vi "Remove Buffer.vi"(8 "error in":errorcluster, 9 "Name":string, 11 "BufferMap in":refnum<data-value>) -> (0 "error out":errorcluster, 2 "Buffer":refnum<data-value>, 3 "BufferMap":refnum<data-value>)   [LabVIEW 2013, in "CircularBuffer.lvlib" / "VariantBufferMap.lvclass"]
doc: "This VI writes one data element into the current location in the buffer. The location in the buffer is updated automatically."
uses:
  VariantBufferMap.lvclass
  VariantBuffer/VariantBuffer.lvclass
  VariantBufferMap.lvclass/VariantBufferMap.ctl
  VariantBuffer/WriteBufferError.vi
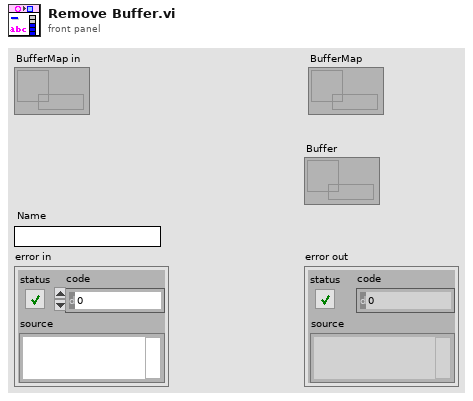
[diagram p1: front panel]
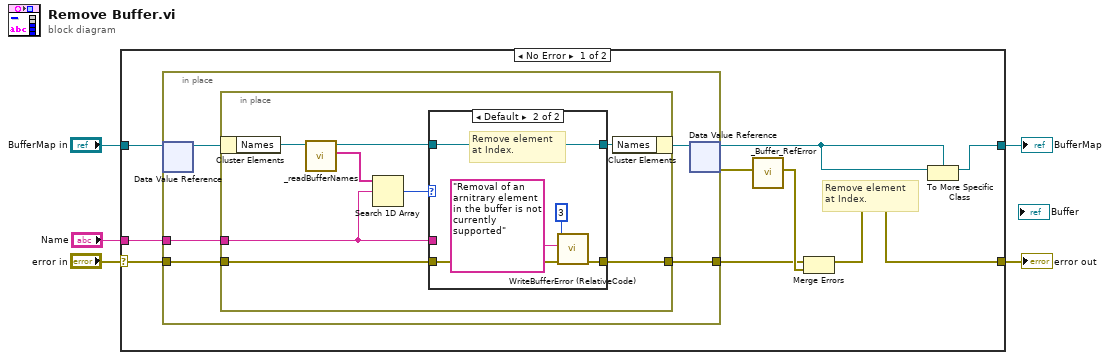
[diagram p0: block diagram]
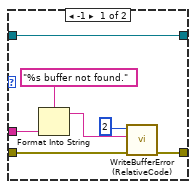
[diagram p2: hidden frame]
diagram:
  n1 = case shown="No Error" "error in" {
    selector: "error in" -> [w9 w41]
    tunnel: "BufferMap in" -> [w12 w40]
    tunnel: [w13 w40] -> w4
    tunnel: [w6 w41] -> w3
    tunnel: "Name" -> [w14 _]
    frame No Error {
      # "Remove element \nat Index."
      n2 = in-place {
        in-place-border: w14 -> [w17]
        in-place-border: [w16] -> w8
        in-place-border: w9 -> [w15]
        n3 = in-place-dvr #1(w12) -> (w19:refnum<class "VariantBufferMap.lvclass">)  [unwired: 1 out]
        n4 = in-place {
          in-place-border: w17 -> [w25]
          in-place-border: [w24] -> w16
          in-place-border: w15 -> [w20]
          n5 = in-place-cluster #2(w19) -> ("Names"=w27:refnum<data-value>)
          n6 = call "_readBufferNames.vi"("Data Value Reference in"=w27) -> ("Names"=w23:string[], "Data Value Reference out"=w21:refnum<data-value>)  [unwired: 9 in]
          n7 = Search 1D Array(1D array=w23, element=w25) -> (index of element=w22:i32)  [unwired: 1 in]
          n8 = case shown="Default" w22 {
            tunnel: w21 -> [w34 w39]
            tunnel: [w34 w39] -> w26
            tunnel: w25 -> [w30 _]
            tunnel: [w33 w37] -> w24
            tunnel: w20 -> [w31 w38]
            frame -1 {
              n9 = Format Into String(format string="%s buffer not found." ("error message (\"\")"), w30) -> (resulting string=w29:string)  [unwired: 2 in, 1 out]
              n10 = call "WriteBufferError (RelativeCode).vi"("error in (no error)"=w31, "Error message"=w29, "Relative error code (548600 + input)"=2 ("error code (0)")) -> ("error out"=w33:errorcluster)  [unwired: 8 in]
            }
            frame Default {
              # "Remove element \nat Index."
              n11 = call "WriteBufferError (RelativeCode).vi"("error in (no error)"=w38, "Error message"="Removal of an arnitrary element in the buffer is not currently supported" ("error message (\"\")"), "Relative error code (548600 + input)"=3) -> ("error out"=w37:errorcluster)  [unwired: 8 in]
            }
          }
          n12 = in-place-cluster #2("Names"=w26) -> (w18:refnum<class "VariantBufferMap.lvclass">)
        }
        n13 = in-place-dvr #1(w18) -> (w7:refnum<data-value>, w11:errorcluster)
      }
      n14 = call "_Buffer_RefError.vi"("error in (no error)"=w11) -> ("error out"=w10:errorcluster)  [unwired: 10 in]
      n15 = Merge Errors(w8, w10) -> (w6:errorcluster)
      n16 = To More Specific Class(target class=w7, reference=w7) -> (specific class reference=w13:refnum<data-value>)  [unwired: 1 in, 1 out]
    }
    frame Error {
    }
  }
  "error out" <- w3
  "BufferMap" <- w4
